vi "Create Server Library from Template.vi"(8 "error in (no error)":errorcluster, 9 "Generated Server Name":string="Generated Server", 10 "Target Project Path":path, 11 "Application ref in":refnum<vi>) -> (0 "error out":errorcluster, 3 "Server library":refnum<vi>)   [LabVIEW 2019, in "gRPC Template Creation Utility.lvlib"]
uses:
  gRPC Template Creation Utility.lvlib
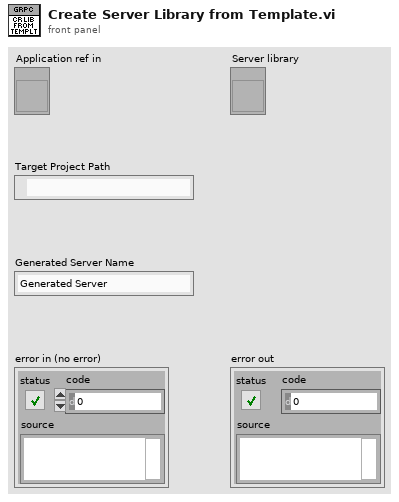
[diagram p1: front panel]
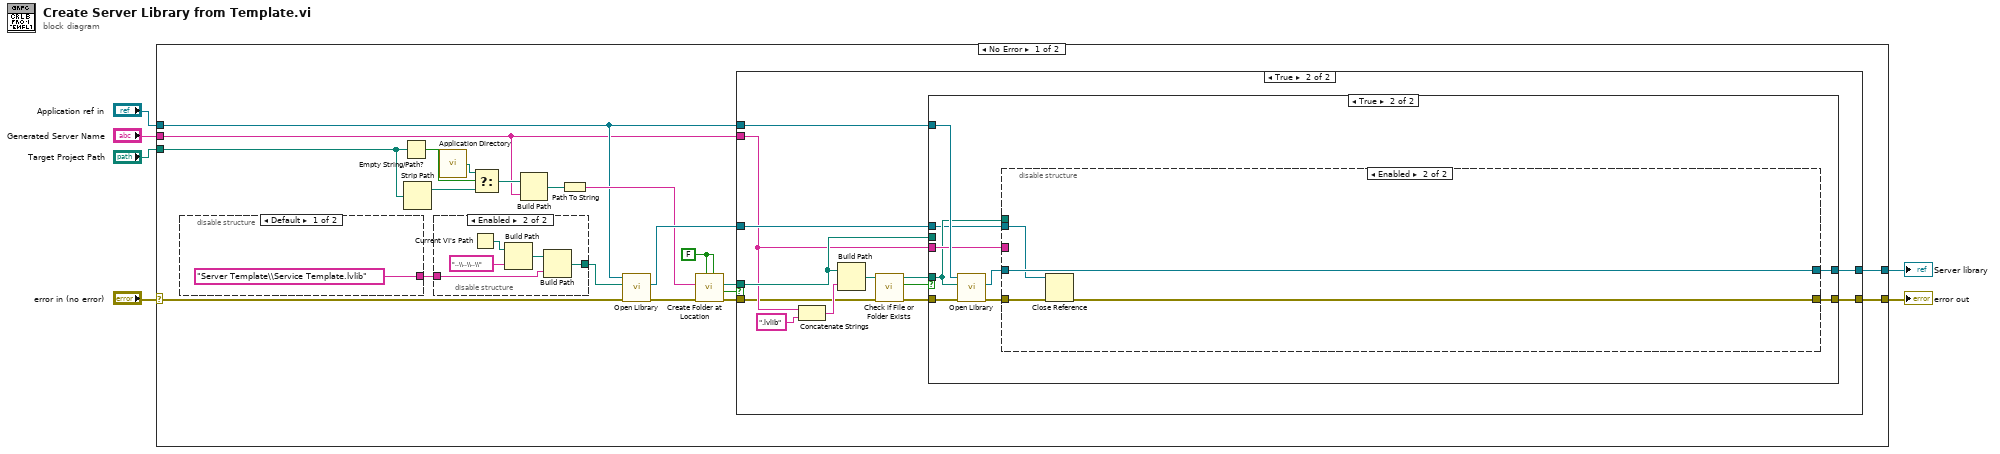
[diagram p0: block diagram]
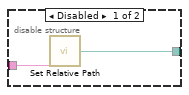
[diagram p2: hidden frame]
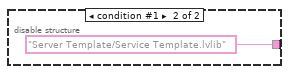
[diagram p3: hidden frame]
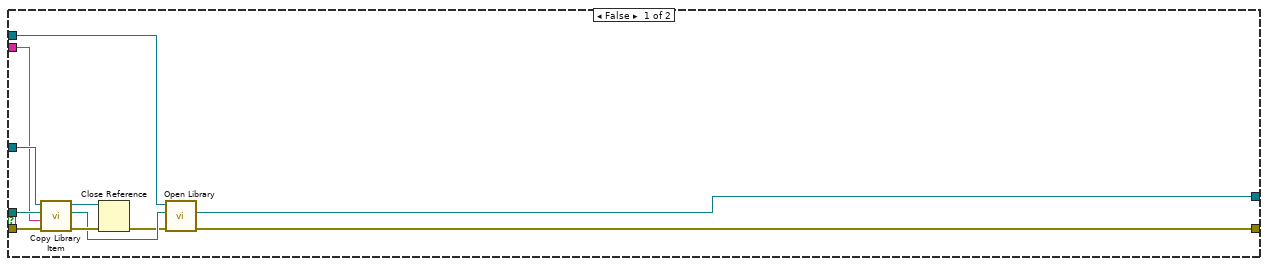
[diagram p4: hidden frame]
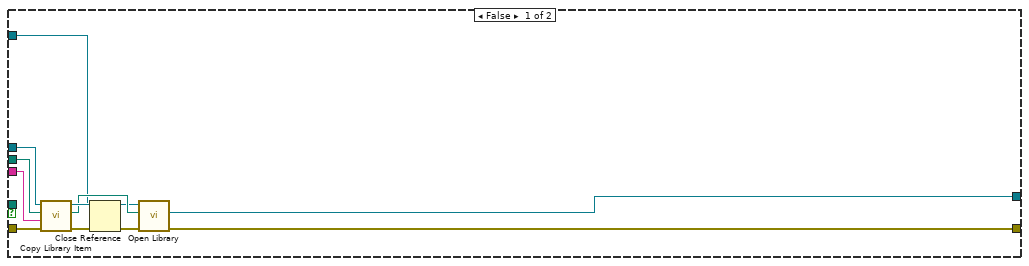
[diagram p5: hidden frame]
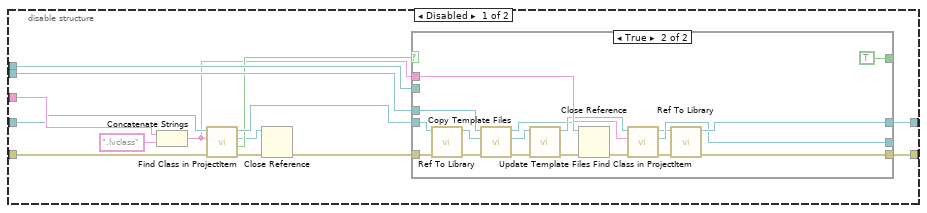
[diagram p6: hidden frame]
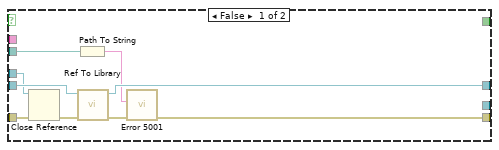
[diagram p7: hidden frame]
diagram:
  n1 = case shown="No Error" "error in (no error)" {
    selector: "error in (no error)" -> [w10 w125]
    tunnel: [w26 w125] -> w6
    tunnel: [w25 _] -> w5
    tunnel: "Target Project Path" -> [w12 _]
    tunnel: "Generated Server Name" -> [w7 _]
    tunnel: "Application ref in" -> [w11 _]
    frame No Error {
      w19 = FALSE ("Use Relative")
      n2 = disable-structure shown="Default" {
        disable-tunnel: ["Server Template\\Service Template.lvlib" ("Application Relative Path") "Server Template/Service Template.lvlib" ("Application Relative Path")] -> w8
        frame condition #0 (active) {
        }
        frame condition #1 {
        }
      }
      n3 = Empty String/Path?(string/path=w12) -> (empty?=w16:bool)
      n4 = Strip Path(path=w12) -> (stripped path=w15:path)  [unwired: 1 out]
      n5 = disable-structure shown="Enabled" {
        disable-tunnel: [w28 w31] -> w22
        disable-tunnel: w8 -> [w27 w29]
        frame Disabled {
          n6 = call "Set Relative Path.vi"("Application Relative Path"=w27) -> ("Full Path"=w28:path)
        }
        frame Enabled {
          n7 = Current VI's Path() -> (path=w33:path)
          n8 = Build Path(base path=w33, name or relative path="..\\..\\..\\") -> (appended path=w30:path)
          n9 = Build Path(base path=w30, name or relative path=w29) -> (appended path=w31:path)
        }
      }
      n10 = call <vilib>:"Application Directory.vi"() -> ("Application Directory"=w13:path)
      n11 = Select(t=w13, s=w16, f=w15) -> (s? t:f=w14:path)
      n12 = Build Path(base path=w14, name or relative path=w7) -> (appended path=w18:path)
      n13 = Path To String(path=w18) -> (string=w17:string)
      n14 = call "Open Library.vi"("error in (no error)"=w10, "Full Path"=w22, "Application in"=w11) -> ("error out"=w23:errorcluster, "Library out"=w20:refnum<vi>)  [unwired: 6 in, 1 out]
      n15 = call "Create Folder at Location.vi"("Override existing (F)"=w19, "Use Relative (F)"=w19, "Error In"=w23, "Path"=w17) -> ("Error Out"=w24:errorcluster, "Already Exists ?"=w9:bool, "Full path out"=w21:path)  [unwired: 5 in]
      n16 = case shown="True" w9 {
        tunnel: [w38 w50] -> w26
        tunnel: [w46 w55] -> w25
        tunnel: w24 -> [w43 w48]
        tunnel: w21 -> [w42 w52]
        tunnel: w20 -> [w41 w53]
        tunnel: w7 -> [w37 w51]
        tunnel: w11 -> [w36 w54]
        frame False {
          n17 = call "Copy Library Item.vi"("error in (no error)"=w43, "Copy Name"=w37, "Copy location"=w42, "Library in"=w41) -> ("error out"=w45:errorcluster, "New Lib Path"=w40:path, "Library out"=w44:refnum<vi>)  [unwired: 5 in]
          n18 = Close Reference(reference=w44, error in (no error)=w45) -> (error out=w39:errorcluster)
          n19 = call "Open Library.vi"("error in (no error)"=w39, "Full Path"=w40, "Application in"=w36) -> ("error out"=w38:errorcluster, "Library out"=w46:refnum<vi>)  [unwired: 6 in, 1 out]
        }
        frame True {
          n20 = Concatenate Strings(w51, ".lvlib" ("string")) -> (w58:string)
          n21 = Build Path(base path=w52, name or relative path=w58) -> (appended path=w57:path)
          n22 = call <vilib>:"Check if File or Folder Exists.vi"("error in (no error)"=w48, "path"=w57) -> ("error out"=w47:errorcluster, "file or folder exists?"=w56:bool, "dup path"=w49:path)  [unwired: 7 in]
          n23 = case shown="True" w56 {
            tunnel: [w65 w77] -> w55
            tunnel: w54 -> [w64 w79]
            tunnel: w53 -> [w63 w74]
            tunnel: w52 -> [w62 _]
            tunnel: w51 -> [w61 w78]
            tunnel: w47 -> [w60 w73]
            tunnel: [w66 w76] -> w50
            tunnel: w49 -> [_ w75]
            frame False {
              n24 = call "Copy Library Item.vi"("error in (no error)"=w60, "Copy Name"=w61, "Copy location"=w62, "Library in"=w63) -> ("error out"=w70:errorcluster, "New Lib Path"=w68:path, "Library out"=w69:refnum<vi>)  [unwired: 5 in]
              n25 = Close Reference(reference=w69, error in (no error)=w70) -> (error out=w67:errorcluster)
              n26 = call "Open Library.vi"("error in (no error)"=w67, "Full Path"=w68, "Application in"=w64) -> ("error out"=w66:errorcluster, "Library out"=w65:refnum<vi>)  [unwired: 6 in, 1 out]
            }
            frame True {
              n27 = call "Open Library.vi"("error in (no error)"=w73, "Full Path"=w75, "Application in"=w79) -> ("error out"=w71:errorcluster, "Library out"=w72:refnum<vi>)  [unwired: 6 in, 1 out]
              n28 = disable-structure shown="Enabled" {
                disable-tunnel: w78 -> [w93 _]
                disable-tunnel: [w92 w124] -> w77
                disable-tunnel: [w91 w121] -> w76
                disable-tunnel: w75 -> [w90 _]
                disable-tunnel: w74 -> [w89 w123]
                disable-tunnel: w72 -> [w88 w124]
                disable-tunnel: w71 -> [w86 w122]
                frame Disabled {
                  n29 = Concatenate Strings(w93, ".lvclass" ("Class Name")) -> (w80:string)
                  n30 = call "Find Class in ProjectItem.vi"("error in (no error)"=w86, "Class Name"=w80, "ProjectItem in"=w88) -> ("error out"=w82:errorcluster, "Found?"=w84:bool, "LVClass out"=w83:refnum<vi>, "ProjectItem out"=w85:refnum<vi>)  [unwired: 5 in]
                  n31 = Close Reference(reference=w83, error in (no error)=w82) -> (error out=w81:errorcluster)
                  n32 = case shown="True" w84 {
                    tunnel: w85 -> [w102 w115]
                    tunnel: [w101 w120] -> w92
                    tunnel: w81 -> [w96 w117]
                    tunnel: [w99 w108] -> w91
                    tunnel: w90 -> [w98 _]
                    tunnel: [_ TRUE] -> _
                    tunnel: w89 -> [w97 w107]
                    tunnel: w80 -> [_ w114]
                    tunnel: [_ w113] -> _
                    frame False {
                      n33 = Close Reference(reference=w97, error in (no error)=w96) -> (error out=w95:errorcluster)
                      n34 = Path To String(path=w98) -> (string=w94:string)
                      n35 = call "Ref To Library.vi"("error in (no error)"=w95, "ProjectItem in"=w102) -> ("error out"=w100:errorcluster, "Library out"=w101:refnum<vi>)  [unwired: 8 in]
                      n36 = call "Error 5001.vi"("error in (no error)"=w100, "Server Class Path"=w94) -> ("error out"=w99:errorcluster)  [unwired: 9 in]
                    }
                    frame True {
                      n37 = call "Ref To Library.vi"("error in (no error)"=w117, "ProjectItem in"=w115) -> ("error out"=w116:errorcluster, "Library out"=w118:refnum<vi>)  [unwired: 8 in]
                      n38 = call "Copy Template Files.vi"("error in (no error)"=w116, "Server Library (Library Item) in"=w118, "Template Library (Library Item) in"=w107) -> ("error out"=w106:errorcluster, "Server Library (Library Item) out"=w105:refnum<vi>, "Template Library (Library Item) out"=w103:refnum<vi>)  [unwired: 6 in]
                      n39 = call "Update Template Files.vi"("error in (no error)"=w106, "Server Library (Library Item) in"=w105) -> ("error out"=w104:errorcluster, "Server Library (Library Item) out"=w112:refnum<vi>)  [unwired: 8 in]
                      n40 = Close Reference(reference=w103, error in (no error)=w104) -> (error out=w110:errorcluster)
                      n41 = call "Find Class in ProjectItem.vi"("error in (no error)"=w110, "Class Name"=w114, "ProjectItem in"=w112) -> ("error out"=w109:errorcluster, "LVClass out"=w113:refnum<vi>, "ProjectItem out"=w111:refnum<vi>)  [unwired: 5 in, 1 out]
                      n42 = call "Ref To Library.vi"("error in (no error)"=w109, "ProjectItem in"=w111) -> ("error out"=w108:errorcluster, "Library out"=w120:refnum<vi>)  [unwired: 8 in]
                    }
                  }
                }
                frame Enabled {
                  n43 = Close Reference(reference=w123, error in (no error)=w122) -> (error out=w121:errorcluster)
                }
              }
            }
          }
        }
      }
    }
    frame Error {
    }
  }
  "error out" <- w6
  "Server library" <- w5
